vi "VarMan Spy.vi"() -> ()   [LabVIEW 2021]
doc: "VarMan Spy monitors VarMan's objects and allows performing some manipulations on them. Use a \"Spy\" menu to control the Spy.\nFor more information, see online help for the Spy.\n\n::: CalcExpress Toolkit :::\nCopyright (c) 2000-2026 Konstantin Shifershteyn. All rights reserved."
uses:
  _VarMan Spy.llb/VM Spy Type - Display Mode Selector.ctl
  <vilib>/Utility/sysdir.llb/System Directory Type.ctl
  <vilib>/Utility/miscctls.llb/LVRowAndColumnUnsignedTypeDef.ctl
  vi.lib/addons/CalcExpress/cemisc.llb/[ce] CE component paths - Kind of Path Enum.ctl
  <vilib>/Utility/config.llb/NI_LVConfig.lvlib
panel:
  in  "EnaFilter":bool=TRUE caption="Name filter"
  in  "NamePtrn":string caption="Name pattern"
  in  "VarList Mode":T1 caption="Display mode"
  in  "VC List":i32(listbox)=-1 caption="Context List"
  out "ctx info line":string caption="Context creator"
  in  "MaxWriteTS":dbl
  in  "Var List":i32[](listbox) caption="Variable List"
  out "var info line":string caption="info line"
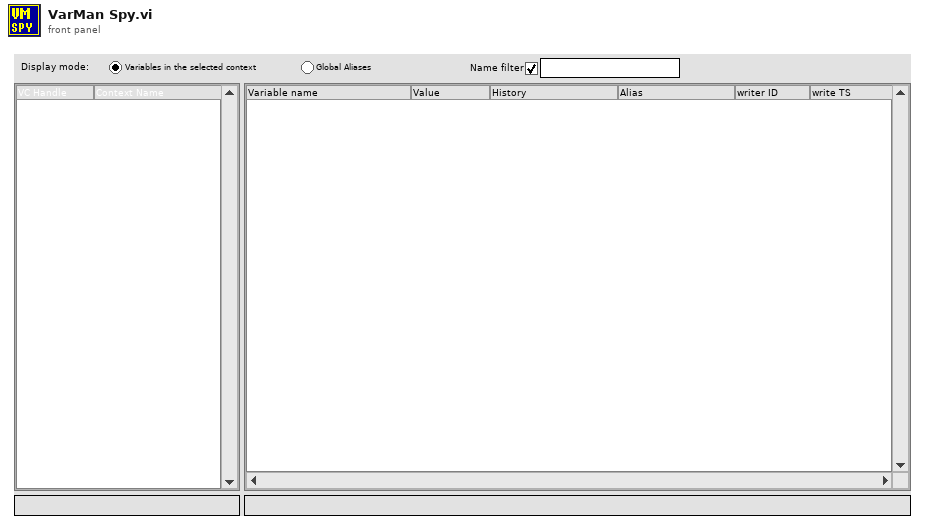
[diagram p1: front panel]
types:
  T1 = typedef "VM Spy Type - Display Mode Selector.ctl" = enum32{"Variables", "Aliases"}
  T2 = typedef "System Directory Type.ctl" = i32
  T3 = enum32{"invalid OS target", "Mac OS", "Windows 3.1", "Windows 95/NT", "Solaris 1", "Solaris 2", "HP-UX", "PowerMAX", "Linux", "Irix", "Rhapsody", "BeOS", "AIX", "OSF1", "VxWorks", "PharLap", "Carbon", "RTX", "Windows x64", "Linux x64", "Mac OS X x64"}
  T4 = typedef "LVRowAndColumnUnsignedTypeDef.ctl" = cluster{"Row":u32, "Column":u32}
  T5 = enum16{"don't sort", "alias", "vc handle", "name", "type"}
  T6 = typedef "VarMan Variable Context Handle.ctl" = i32
  T7 = typedef "VarMan Variable Info Cluster.ctl" = cluster{"name":string, "alias":string, "type":u32, "history":bool}
  T8 = cluster{"dup VC Handle":T6, "variables info":T7[]}
  T9 = typedef "VarMan Variable Data Statistics.ctl" = cluster{"writer ID":u32, "write MS":u32, "write TS":dbl, "write Cnt":u32}
  T10 = typedef "VarMan Alias Info Cluster.ctl" = cluster{"alias":string, "vc handle":T6, "var name":string, "type":u32, "history":bool}
  T11 = enum32{"invalid app kind", "Development System", "Run Time System", "Student Edition", "Embedded LabVIEW", "Evaluation", "Custom"}
  T12 = enum32{"Invalid", "Standard", "Closed", "Hidden", "Minimized", "Maximized"}
  T13 = typedef "[ce] CE component paths - Kind of Path Enum.ctl" = enum16{"VIs", "FuncVIs", "Help", "Examples", "Project", "Templates"}
  T14 = typedef "eventvkey.ctl" = enum16{"ASCII", "Enter", "Return", "Shift", "Ctrl", "Alt", "Cmd", "Opt", "Caps", "NumLock", "Clear", "Break", "Up", "Down", "Left", "Right", "Insert", "Delete", "Home", "End", "PageUp", "PageDown", "Escape", "Help", "Pause", "ScrollLock", "F1", "F2", "F3", "F4", "F5", "F6", "F7", "F8", "F9", "F10", "F11", "F12", "F13", "F14", "F15", "F16", "F17", "F18", "F19", "F20", "F21", "F22", "F23", "F24", "Play", "VolumeUp", "VolumeDown", "Mute", "Two Byte Char"}
  T15 = cluster{"Shift":bool, "Ctrl":bool, "Alt":bool, "Cmd":bool, "Opt":bool}
  T16 = typedef "LVPoint32TypeDef.ctl" = cluster{"Horizontal":i32, "Vertical":i32}
  T17 = typedef "LVRowAndColumnTypeDef.ctl" = cluster{"Row":i32, "Column":i32}
  T18 = typedef "NI_LVConfig.lvlib/Config Data RefNum.ctl" = refnum<k1>
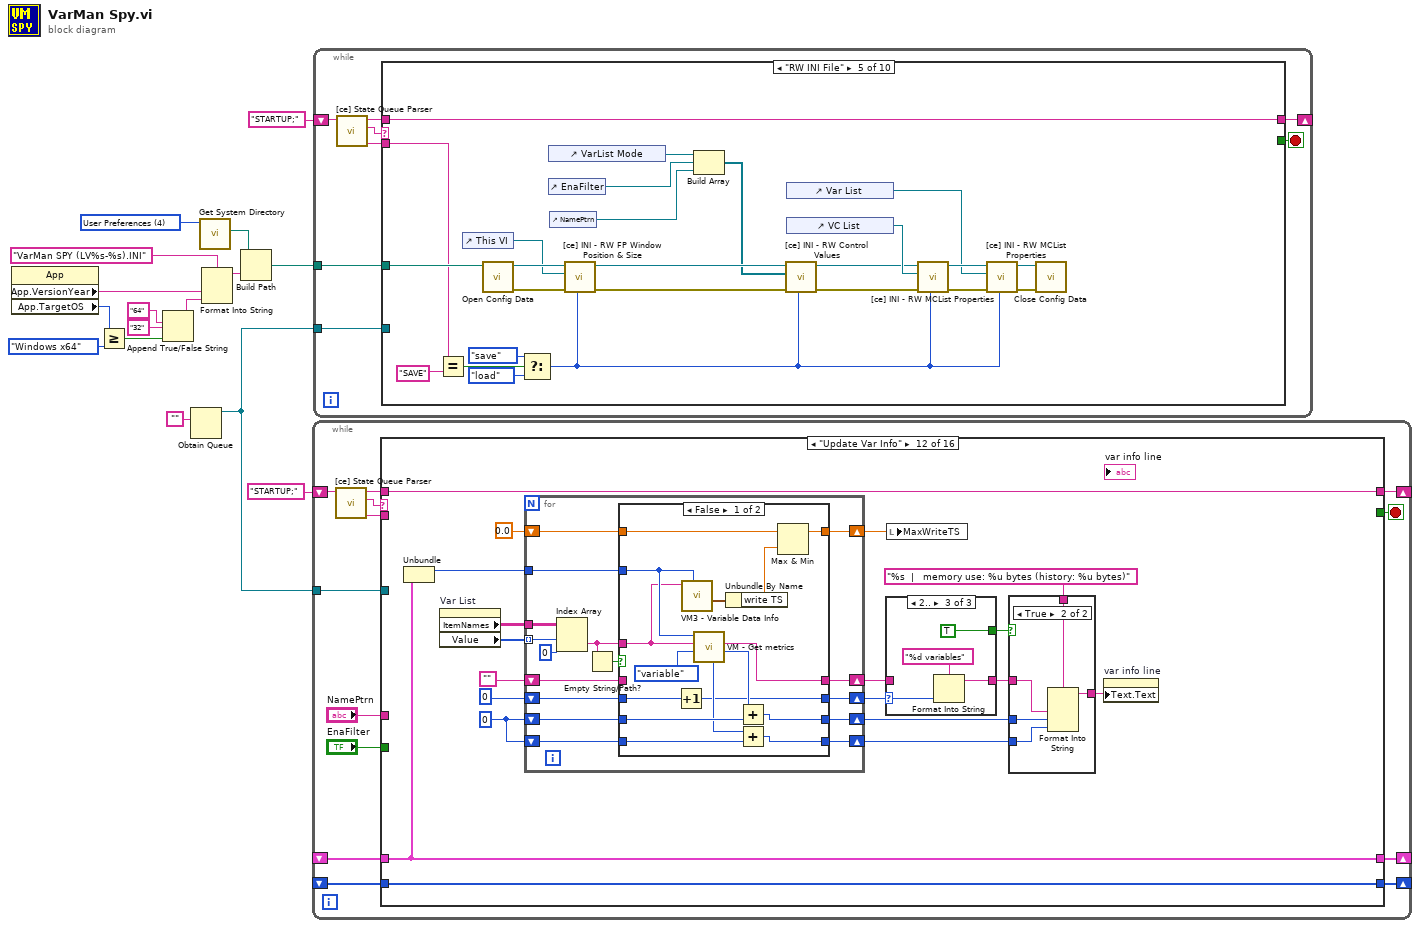
[diagram p0: block diagram]
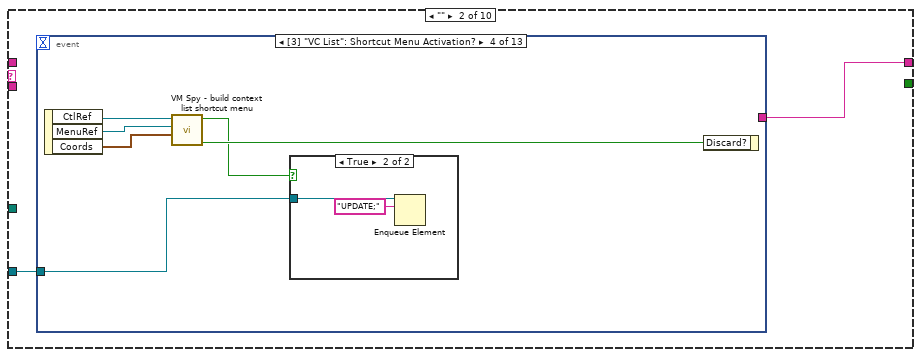
[diagram p3: hidden frame]
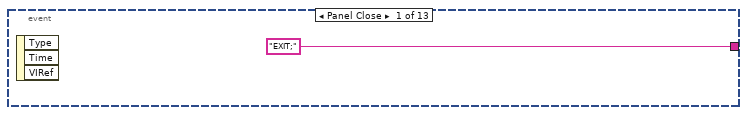
[diagram p4: hidden frame]
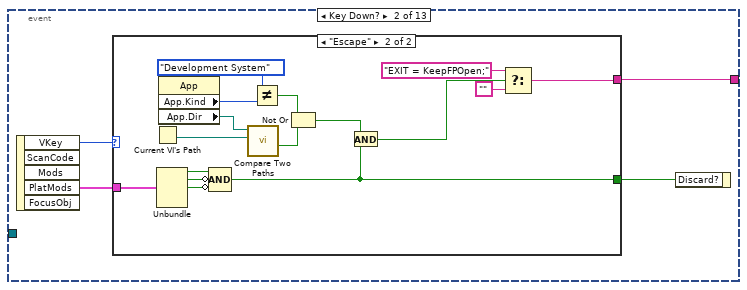
[diagram p5: hidden frame]
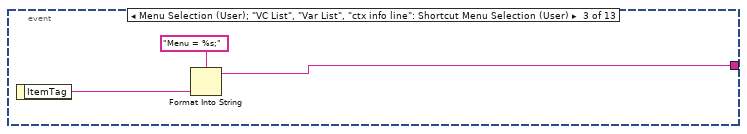
[diagram p7: hidden frame]
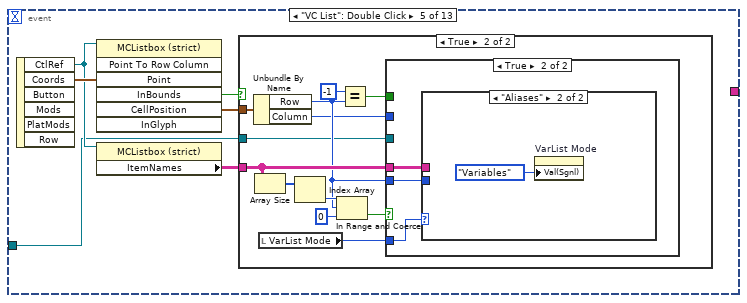
[diagram p9: hidden frame]
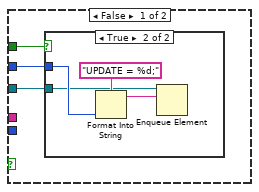
[diagram p11: hidden frame]
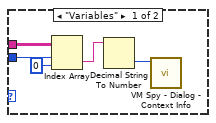
[diagram p13: hidden frame]
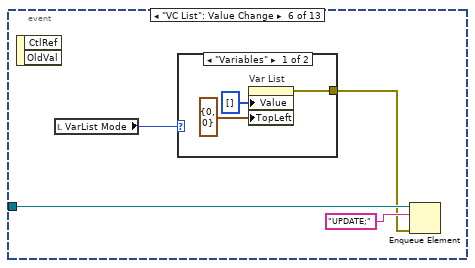
[diagram p14: hidden frame]
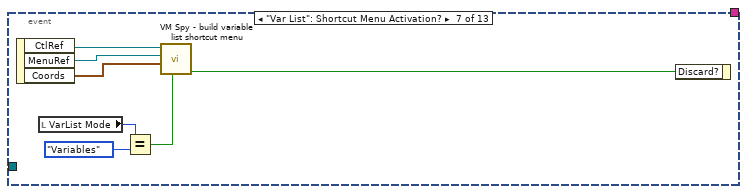
[diagram p16: hidden frame]
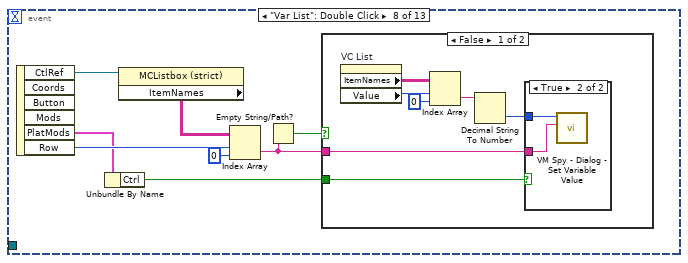
[diagram p17: hidden frame]
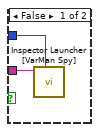
[diagram p18: hidden frame]
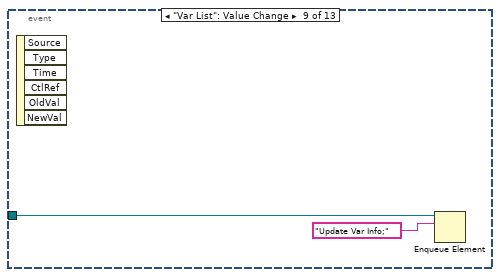
[diagram p20: hidden frame]
diagram:
  w2 = T2 4 items=["User Home"=0, "User Desktop"=1, "User Documents"=2, "User Application Data"=3, "User Preferences"=4, "User Temporary"=5, "Public Documents"=6, "Public Application Data"=7, "Public Preferences"=8, "Public Cache"=13, "System Core Libraries"=9, "System Installed Libraries"=10, "Application Files"=11, "Boot Volume Root"=12] ("system directory type")
  n1 = property class="App"() -> ("App.VersionYear"=w12:string, "App.TargetOS"=w10:T3)  [unwired: 2 in, 2 out]
  n2 = Greater Or Equal?(x=w10, y=T3."Windows x64" ("Application:Target:Operating System")) -> (x >= y?=w11:bool)
  n3 = Append True/False String(1:w11, 2:"32", 3:"64") -> (0:w9:string)  [unwired: 1 in]
  n4 = Obtain Queue(element data type="") -> (queue out=w13:refnum<queue>)  [unwired: 4 in, 2 out]
  n5 = call <vilib>:"Get System Directory.vi"("system directory type"=w2) -> ("system directory"=w8:path)  [unwired: 10 in]
  n6 = Format Into String(format string="VarMan SPY (LV%s-%s).INI", w12, w9) -> (resulting string=w7:string)  [unwired: 2 in, 1 out]
  n7 = Build Path(base path=w8, name or relative path=w7) -> (appended path=w1:path)
  n8 = while {
    shift-right: [w27] -> _
    shift-left: "STARTUP;" -> [w28]
    tunnel: w13 -> [w24]
    shift-right: [w21] -> _
    shift-left: _ -> [w20]
    shift-right: [w22] -> _
    shift-left: _ -> [w19]
    stop <- w25 stop-if-true
    n9 = call "[ce] State Queue Parser.vi"("input queue"=w28) -> ("state parameters"=w23:string, "state"=w29:string, "remained queue"=w26:string)  [unwired: 6 in]
    n10 = case shown="\"Update Var Info\"" w29 {
      tunnel: [w32 w43 w54 w59 w64 w71 w74 w98 w126 w142 w280 w385 w441 w444 w453 w457] -> w27
      tunnel: w26 -> [w32 _ w55 w60 w65 w71 w74 w99 w126 w149 w290 w385 w441 w444 w453 w464]
      tunnel: [_ _ _ _ _ TRUE _ _ _ _ _ _ _ _ _ _] -> w25
      tunnel: w24 -> [_ w50 _ _ _ w66 _ _ _ _ _ _ _ _ _ _]
      tunnel: w23 -> [_ _ _ _ _ _ _ w94 w117 w134 w272 _ _ _ w449 w460]
      tunnel: [w31 w34 w52 w57 w62 w69 w73 w97 w114 w147 w288 w382 w439 w443 w454 w465] -> w22
      tunnel: [w30 w33 w51 w56 w61 w68 w72 w96 w113 w148 w289 w384 w440 w442 w455 w459] -> w21
      tunnel: w20 -> [w30 w33 w51 w56 w61 w68 w72 w96 w112 w148 w289 w384 w440 w442 w455 w459]
      tunnel: w19 -> [w31 w34 w52 w57 w62 w69 w73 w97 _ w147 w288 w382 w439 w443 w454 w465]
      tunnel: "NamePtrn" -> [_ _ _ _ _ _ _ _ _ w132 w270 _ _ _ _ _]
      tunnel: "EnaFilter" -> [_ _ _ _ _ _ _ _ _ w131 w264 _ w438 _ _ _]
      frame Default {
      }
      frame "" {
        n11 = Dequeue Element(queue=w50, timeout in ms (-1)=100) -> (element=w47:string, error out=w46:errorcluster)  [unwired: 1 in, 2 out]
        n12 = Tick Count (ms)() -> (millisecond timer value=w42:u32)
        n13 = Quotient & Remainder(x=w42, y=u32 500) -> (floor(x/y)=w39:u32)  [unwired: 1 out]
        n14 = feedback-in #1(w39) -> ()
        n15 = feedback #1() -> (w40:u32)  [unwired: 1 in]
        n16 = Not Equal?(x=w39, y=w40) -> (x != y?=w38:bool)
        n17 = Select(t="UPDATE;", s=w38, f="") -> (s? t:f=w35:string)
        n18 = Empty String/Path?(string/path=w47) -> (empty?=w48:bool)
        n19 = Select(t=w35, s=w48, f=w47) -> (s? t:f=w45:string)
        n20 = Select(t="EXIT;", s=w46, f=w45) -> (s? t:f=w43:string)
      }
      frame "STARTUP" {
        n21 = Concatenate Strings("INIT;", w55) -> (w54:string)
      }
      frame "INIT" {
        n22 = Concatenate Strings("", w60) -> (w59:string)
      }
      frame "EXIT" {
        n23 = Concatenate Strings("HALT;", w65) -> (w64:string)
      }
      frame "HALT" {
        n24 = Release Queue(queue=w66, force destroy? (F)=TRUE) -> ()  [unwired: 1 in, 3 out]
      }
      frame "------------------------------------ 1" {
      }
      frame "UPDATE" {
        n25 = feedback-in #2("VarList Mode") -> ()
        n26 = feedback #2() -> (w93:T1)  [unwired: 1 in]
        n27 = First Call?() -> (First Call?: T/F=w91:bool)
        n28 = Not Equal?(x="VarList Mode", y=w93) -> (x != y?=w92:bool)
        n29 = Or(x=w92, y=w91) -> (x .or. y?=w90:bool)
        n30 = case shown="True" w90 {
          tunnel: "VarList Mode" -> [_ w103]
          tunnel: [_ TRUE] -> w88
          frame False {
          }
          frame True {
            n31 = case shown="\"Variables\"" w103 {
              tunnel: [string[] ["Variable name", "Value", "History", "Alias", "writer ID", "write TS"] ("Column Header Strings[]") string[] ["Alias", "Value", "History", "Variable", "writer ID", "write TS"] ("Column Header Strings[]")] -> w104
              frame "Variables" {
              }
              frame "Aliases" {
              }
            }
            n32 = property on="Var List" class="MCListbox (strict)"("ColHdrString"=w104, "TopLeft"=T4 {"Row"=0, "Column"=0} ("Top Left Visible Cell"), "Value"=i32[] [] ("Var List")) -> ()  [unwired: 2 in, 2 out]
          }
        }
        n33 = case shown="\"Aliases\"" "VarList Mode" {
          tunnel: ["Update Var List = %s;" "Update Alias List = %s;"] -> w79
          frame "Variables" {
          }
          frame "Aliases" {
          }
        }
        n34 = Format Into String(format string="Update VC List = %s;", w94) -> (resulting string=w81:string)  [unwired: 2 in, 1 out]
        n35 = feedback #3(u32 0) -> (w86:u32)
        n36 = Increment(x=w86) -> (x+1=w84:u32)
        n37 = feedback-in #3(w84) -> ()
        n38 = Quotient & Remainder(x=w84, y=u32 20) -> (x-y*floor(x/y)=w82:u32)  [unwired: 1 out]
        n39 = Equal To 0?(x=w82) -> (x = 0?=w87:bool)
        n40 = Or(x=w87, y=w88) -> (x .or. y?=w78:bool)
        n41 = Select(t="MAX", s=w78, f="") -> (s? t:f=w76:string)
        n42 = Format Into String(format string=w79, w76) -> (resulting string=w80:string)  [unwired: 2 in, 1 out]
        n43 = Concatenate Strings(w81, w80, w99) -> (w98:string)
      }
      frame "Update VC List" {
        n44 = Decimal String To Number(string=w117, default (0L)=-1 ("default (0 I32)")) -> (number=w115:i32)  [unwired: 1 in, 1 out]
        n45 = control-ref of="VC List"() -> (w120:refnum<vi>)
        n46 = Index Array(array=w112, index="VC List") -> (element=w122:T6)
        n47 = call "VM Spy - build list of contexts.vi"("sort column"=w115, "MCListbox Refnum"=w120) -> ("array of VC handles"=w113:T6[], "dup MCListbox Refnum"=w119:refnum<vi>)  [unwired: 5 in, 1 out]
        n48 = Search 1D Array(1D array=w113, element=w122) -> (index of element=w121:i32)  [unwired: 1 in]
        n49 = Not Equal?(x=w121, y="VC List") -> (x != y?=w123:bool)
        n50 = Index Array(array=w113, index=w121) -> (element=w118:T6)
        n51 = case shown="True" w123 {
          tunnel: w121 -> [_ w128]
          tunnel: w119 -> [_ w127]
          frame False {
          }
          frame True {
            n52 = local write "VC List"(w128) -> ()
            n53 = call "VM Spy - MCListBox make row visible.vi"("visible row"=w128, "MCListbox Refnum"=w127) -> ()  [unwired: 6 in, 2 out]
          }
        }
        n54 = call "VM - Context Info.vi"("VC Handle"=w118) -> ("Creator"=→"ctx info line":string)  [unwired: 6 in, 4 out]
        n55 = call "VM - List of Variables.vi"("sort"=enum16{"don't sort", "name", "alias", "type"}."name", "VC Handle"=w118) -> ("variables info"=w125:T7[], "dup VC Handle"=w124:T6)  [unwired: 5 in, 1 out]
        n56 = Bundle("dup VC Handle"=w124, "variables info"=w125) -> (w114:T8)  [unwired: 1 in]
      }
      frame "Update Var List" {
        n57 = Unbundle(w147) -> ("dup VC Handle"=w143:T6, "variables info"=w137:T7[])
        n58 = Empty String/Path?(string/path=w132) -> (empty?=w133:bool)
        n59 = Compound Arithmetic op=OR(w133, invert w131) -> (w130:bool)
        n60 = for {
          tunnel: w137 -> [w193] mode=indexing
          tunnel: w143 -> [w189]
          tunnel: [w191] -> w146 mode=indexing if=w185
          tunnel: [w190] -> w145 mode=indexing if=w185
          tunnel: [w187] -> w138 mode=indexing if=w185
          tunnel: w132 -> [w182]
          tunnel: w130 -> [w181]
          n61 = Unbundle By Name(w193) -> ("alias"=w184:string, "history"=w188:bool, "name"=w183:string, "type"=w192:u32)
          n62 = case shown="False" w181 {
            selector: w181 -> [_ w198]
            tunnel: [w196 w198] -> w186
            tunnel: w183 -> [w195 _]
            tunnel: w182 -> [w194 _]
            frame False {
              n63 = Match Pattern(string=w195, regular expression=w194) -> (offset past match=w197:i32)  [unwired: 1 in, 3 out]
              n64 = Greater Or Equal To 0?(x=w197) -> (x >= 0?=w196:bool)
            }
            frame True {
            }
          }
          n65 = case shown="True" w186 {
            tunnel: w192 -> [_ w215]
            tunnel: w184 -> [_ w213]
            tunnel: [_ w212] -> w191
            tunnel: [_ w211] -> w190
            tunnel: w189 -> [_ w210]
            tunnel: w183 -> [_ w209]
            tunnel: w188 -> [_ w204]
            tunnel: [_ w200] -> w187
            tunnel: [_ TRUE] -> w185
            frame False {
            }
            frame True {
              n66 = case shown="1" w215 {
                selector: w215 -> [_ _ _ _ _ _ w258]
                tunnel: w209 -> [w219 w226 w233 w236 w244 w249 w253]
                tunnel: w210 -> [w217 w225 w232 w235 w242 w248 w252]
                tunnel: ["..." w222 w229 w238 "[..]" "[[..]]" w260] -> w214
                tunnel: [w218 w224 w231 w240 w243 w247 w261] -> w205
                tunnel: [w216 w221 w227 w234 w241 w246 w251] -> w206
                frame Default {
                  n67 = call "VM3 - Variable Data Info.vi"("VC Handle"=w217, "name_spec"=w219) -> ("stats"=w216:T9, "dup name_spec"=w218:string)  [unwired: 4 in, 4 out]
                }
                frame 0 {
                  n68 = call "VM3 - String.vi"("VC Handle"=w225, "name_spec"=w226) -> ("stats"=w221:T9, "value out"=w223:string, "dup name_spec"=w224:string)  [unwired: 6 in, 1 out]
                  n69 = call "VM Spy - Truncate string value for list.vi"("String in"=w223) -> ("String out"=w222:string)  [unwired: 10 in]
                }
                frame 1 {
                  n70 = call "VM3 - DBL Scalar.vi"("VC Handle"=w232, "name_spec"=w233) -> ("stats"=w227:T9, "value out"=w230:dbl, "dup name_spec"=w231:string)  [unwired: 6 in, 1 out]
                  n71 = Format Value(format string="%.;%#_9g", value (0)=w230) -> (output string=w229:string)  [unwired: 1 in]
                }
                frame 5 {
                  n72 = call "VM3 - CDB Scalar.vi"("VC Handle"=w235, "name_spec"=w236) -> ("stats"=w234:T9, "value out"=w239:cdb, "dup name_spec"=w240:string)  [unwired: 6 in, 1 out]
                  n73 = Format Value(format string="%.;%#_g", value (0)=w239) -> (output string=w238:string)  [unwired: 1 in]
                }
                frame 3, 6, 8 {
                  n74 = call "VM3 - Variable Data Info.vi"("VC Handle"=w242, "name_spec"=w244) -> ("stats"=w241:T9, "dup name_spec"=w243:string)  [unwired: 4 in, 4 out]
                }
                frame 4, 7, 9 {
                  n75 = call "VM3 - Variable Data Info.vi"("VC Handle"=w248, "name_spec"=w249) -> ("stats"=w246:T9, "dup name_spec"=w247:string)  [unwired: 4 in, 4 out]
                }
                frame 252 {
                  n76 = call "VM3 - Arbitrary Data.vi"("var type in"=w258, "VC Handle"=w252, "name_spec"=w253) -> ("stats"=w251:T9, "flattened value out"=w257:string, "dup name_spec"=w261:string)  [unwired: 4 in, 2 out]
                  n77 = call "[ce] Index Range from Flattened String.vi"("Flattened string"=w257) -> ("Index Range"=w256:cluster{"Initial index":i32, "Final index":i32})  [unwired: 10 in]
                  n78 = Unbundle(w256) -> ("Initial index"=w254:i32, "Final index"=w255:i32)
                  n79 = Format Into String(format string="{%d:%d}", w254, w255) -> (resulting string=w260:string)  [unwired: 2 in, 1 out]
                }
              }
              n80 = call "VM Spy - VM Datatype to List Symbol.vi"("VarMan Datatype Code"=w215) -> ("List/Tree Symbol"=w211:i32)  [unwired: 10 in]
              n81 = Unbundle By Name(w206) -> ("writer ID"=w207:u32, "write TS"=w200:dbl)
              n82 = call "VM Spy - format history info for variable list.vi"("Has history"=w204, "Variable name"=w205, "VC Handle"=w210) -> ("String out"=w208:string)  [unwired: 8 in]
              n83 = Number To Decimal String(number=w207) -> (decimal integer string=w203:string)  [unwired: 1 in]
              n84 = Format Date/Time String(time format string (%c)="%X%3u %x", seconds (now)=w200) -> (date/time string=w202:string)  [unwired: 1 in]
              n85 = Build Array(w205, w214, w208, w213, w203, w202) -> (w212:string[])
            }
          }
        }
        n86 = feedback-in #4(w143) -> ()
        n87 = feedback #4() -> (w144:T6)  [unwired: 1 in]
        n88 = Not Equal?(x=w143, y=w144) -> (x != y?=w136:bool)
        n89 = case shown="False" w136 {
          tunnel: w146 -> [w154 w169]
          tunnel: w145 -> [w153 w160]
          tunnel: w138 -> [_ w168]
          tunnel: [TRUE w167] -> w135
          tunnel: w134 -> [_ w161]
          frame True {
            n90 = property on="Var List" class="MCListbox (strict)"("TopLeft"=T4 {"Row"=0, "Column"=0} ("Top Left Visible Cell"), "Value"=i32[] [] ("Var List"), "ItemNames"=w154, "ItemSyms"=w153) -> ()  [unwired: 2 in, 2 out]
          }
          frame False {
            n91 = Array Size(array=w160) -> (size(s)=w164:i32)
            n92 = property on="Var List" class="MCListbox (strict)"("ItemNames"=w169, "ItemSyms"=w160) -> ("Value"=w158:i32[])  [unwired: 2 in, 2 out]
            n93 = feedback #5() -> (w163:i32)  [unwired: 1 in]
            n94 = feedback-in #5(w164) -> ()
            n95 = Empty Array?(array=w158) -> (empty?=w157:bool)
            n96 = Not Equal?(x=w164, y=w163) -> (x != y?=w156:bool)
            n97 = Equal?(x=w161, y="MAX") -> (x = y?=w165:bool)
            n98 = And(x=w157, y=w156) -> (x .and. y?=w155:bool)
            n99 = Or(x=w156, y=w165) -> (x .or. y?=w159:bool)
            n100 = case shown="True" w155 {
              frame False {
              }
              frame True {
                n101 = property on="Var List" class="MCListbox (strict)"("TopLeft"=T4 {"Row"=0, "Column"=0} ("Top Left Visible Cell")) -> ()  [unwired: 2 in, 2 out]
              }
            }
            n102 = case shown="False" w159 {
              selector: w159 -> [_ w180]
              tunnel: w158 -> [w174 _]
              tunnel: w168 -> [w173 _]
              tunnel: "MaxWriteTS" -> [w172 _]
              tunnel: [w171 w180] -> w167
              frame False {
                n103 = for {
                  tunnel: w174 -> [w179] mode=indexing
                  tunnel: w173 -> [w178]
                  tunnel: w172 -> [w176]
                  tunnel: [w175] -> w171
                  stop <- w175 stop-if-true
                  n104 = Index Array(array=w178, index=w179) -> (element=w177:dbl)
                  n105 = Greater?(x=w177, y=w176) -> (0:w175:bool)
                }
              }
              frame True {
              }
            }
          }
        }
        n106 = Select(t="Update Var Info;", s=w135, f="") -> (s? t:f=w140:string)
        n107 = Concatenate Strings("Update UI Properties;", w140, w149) -> (w142:string)
      }
      frame "Update Alias List" {
        n108 = Empty String/Path?(string/path=w270) -> (empty?=w265:bool)
        n109 = call "VM - List of Aliases.vi"("sort"=T5."alias") -> ("aliases info"=w282:T10[])  [unwired: 9 in, 1 out]
        n110 = Compound Arithmetic op=OR(w265, invert w264) -> (w263:bool)
        n111 = for {
          tunnel: w282 -> [w315] mode=indexing
          tunnel: [w313] -> w287 mode=indexing if=w307
          tunnel: [w312] -> w271 mode=indexing if=w307
          tunnel: [w308] -> w285 mode=indexing if=w307
          tunnel: w270 -> [w306]
          tunnel: w263 -> [w303]
          n112 = Unbundle By Name(w315) -> ("alias"=w304:string, "history"=w309:bool, "vc handle"=w310:T6, "var name"=w311:string, "type"=w314:u32)
          n113 = case shown="False" w303 {
            selector: w303 -> [_ w366]
            tunnel: w306 -> [w365 _]
            tunnel: [w363 w366] -> w305
            tunnel: w304 -> [w362 _]
            frame False {
              n114 = Match Pattern(string=w362, regular expression=w365) -> (offset past match=w364:i32)  [unwired: 1 in, 3 out]
              n115 = Greater Or Equal To 0?(x=w364) -> (x >= 0?=w363:bool)
            }
            frame True {
            }
          }
          n116 = case shown="True" w305 {
            tunnel: w314 -> [_ w336]
            tunnel: [_ w334] -> w313
            tunnel: [_ w333] -> w312
            tunnel: w311 -> [_ w325]
            tunnel: w304 -> [_ w323]
            tunnel: w310 -> [_ w322]
            tunnel: w309 -> [_ w321]
            tunnel: [_ w317] -> w308
            tunnel: [_ TRUE] -> w307
            frame False {
            }
            frame True {
              n117 = case shown="1" w336 {
                tunnel: w325 -> [w340 w347 w354 w356]
                tunnel: w322 -> [w338 w346 w353 w357]
                tunnel: ["..." w343 w350 w359] -> w335
                tunnel: [w339 w345 w352 w361] -> w324
                tunnel: [w337 w342 w348 w355] -> w326
                frame Default {
                  n118 = call "VM3 - Variable Data Info.vi"("VC Handle"=w338, "name_spec"=w340) -> ("stats"=w337:T9, "dup name_spec"=w339:string)  [unwired: 4 in, 4 out]
                }
                frame 0 {
                  n119 = call "VM3 - String.vi"("VC Handle"=w346, "name_spec"=w347) -> ("stats"=w342:T9, "value out"=w344:string, "dup name_spec"=w345:string)  [unwired: 6 in, 1 out]
                  n120 = call "VM Spy - Truncate string value for list.vi"("String in"=w344) -> ("String out"=w343:string)  [unwired: 10 in]
                }
                frame 1 {
                  n121 = call "VM3 - DBL Scalar.vi"("VC Handle"=w353, "name_spec"=w354) -> ("stats"=w348:T9, "value out"=w351:dbl, "dup name_spec"=w352:string)  [unwired: 6 in, 1 out]
                  n122 = Format Value(format string="%.;%#_9g", value (0)=w351) -> (output string=w350:string)  [unwired: 1 in]
                }
                frame 5 {
                  n123 = call "VM3 - CDB Scalar.vi"("VC Handle"=w357, "name_spec"=w356) -> ("stats"=w355:T9, "value out"=w360:cdb, "dup name_spec"=w361:string)  [unwired: 6 in, 1 out]
                  n124 = Format Value(format string="%.;%#_g", value (0)=w360) -> (output string=w359:string)  [unwired: 1 in]
                }
              }
              n125 = call "VM Spy - VM Datatype to List Symbol.vi"("VarMan Datatype Code"=w336) -> ("List/Tree Symbol"=w333:i32)  [unwired: 10 in]
              n126 = Unbundle By Name(w326) -> ("writer ID"=w327:u32, "write TS"=w317:dbl)
              n127 = Concatenate Strings("=" ("string"), w323) -> (w332:string)
              n128 = call "VM Spy - format history info for variable list.vi"("Has history"=w321, "Variable name"=w324, "VC Handle"=w322) -> ("String out"=w328:string)  [unwired: 8 in]
              n129 = Format Into String(format string=" (VC:%d)", initial string=w324, w322) -> (resulting string=w329:string)  [unwired: 1 in, 1 out]
              n130 = Number To Decimal String(number=w327) -> (decimal integer string=w320:string)  [unwired: 1 in]
              n131 = Format Date/Time String(time format string (%c)="%X%3u %x", seconds (now)=w317) -> (date/time string=w319:string)  [unwired: 1 in]
              n132 = Build Array(w332, w335, w328, w329, w320, w319) -> (w334:string[])
            }
          }
        }
        n133 = Array Size(array=w271) -> (size(s)=w283:i32)
        n134 = property on="Var List" class="MCListbox (strict)"("ItemNames"=w287, "ItemSyms"=w271) -> ("Value"=w267:i32[])  [unwired: 2 in, 2 out]
        n135 = feedback #6() -> (w284:i32)  [unwired: 1 in]
        n136 = feedback-in #6(w283) -> ()
        n137 = local read "MaxWriteTS"() -> (w281:dbl)
        n138 = Empty Array?(array=w267) -> (empty?=w269:bool)
        n139 = Not Equal?(x=w283, y=w284) -> (x != y?=w266:bool)
        n140 = Equal?(x=w272, y="MAX") -> (x = y?=w276:bool)
        n141 = And(x=w269, y=w266) -> (x .and. y?=w268:bool)
        n142 = Or(x=w266, y=w276) -> (x .or. y?=w275:bool)
        n143 = case shown="False" w275 {
          selector: w275 -> [_ w302]
          tunnel: w285 -> [w295 _]
          tunnel: w267 -> [w294 _]
          tunnel: w281 -> [w293 _]
          tunnel: [w292 w302] -> w274
          tunnel: w268 -> [w291 _]
          frame False {
            n144 = case shown="True" w291 {
              frame False {
              }
              frame True {
                n145 = property on="Var List" class="MCListbox (strict)"("TopLeft"=T4 {"Row"=0, "Column"=0} ("Top Left Visible Cell")) -> ()  [unwired: 2 in, 2 out]
              }
            }
            n146 = for {
              tunnel: w294 -> [w301] mode=indexing
              tunnel: w295 -> [w300]
              tunnel: w293 -> [w298]
              tunnel: [w297] -> w292
              stop <- w297 stop-if-true
              n147 = Index Array(array=w300, index=w301) -> (element=w299:dbl)
              n148 = Greater?(x=w299, y=w298) -> (0:w297:bool)
            }
          }
          frame True {
          }
        }
        n149 = Select(t="Update Var Info;", s=w274, f="") -> (s? t:f=w277:string)
        n150 = Concatenate Strings("Update UI Properties;", w277, w290) -> (w280:string)
      }
      frame "Update Var Info" {
        w379 = u64 0
        n151 = Unbundle(w382) -> ("dup VC Handle"=w373:T6)  [unwired: 1 out]
        n152 = property on="Var List" class="MCListbox (strict)"() -> ("ItemNames"=w383:string[][], "Value"=w380:i32[])  [unwired: 2 in, 2 out]
        n153 = for {
          tunnel: w383 -> [w413]
          tunnel: w380 -> [w412] mode=indexing
          shift-right: [w410] -> w378
          shift-left: w379 -> [w409]
          shift-right: [w408] -> w377
          shift-left: w379 -> [w407]
          shift-right: [w404] -> w370
          shift-left: "" -> [w403]
          shift-right: [w402] -> w372
          shift-left: 0 -> [w401]
          tunnel: w373 -> [w400]
          shift-right: [w398] -> w367
          shift-left: 0.0 -> [w399]
          n154 = Index Array(array=w413, index (row)=w412, index (col)=0 ("disabled index (col)")) -> (element=w405:string)
          n155 = Empty String/Path?(string/path=w405) -> (empty?=w406:bool)
          n156 = case shown="False" w406 {
            tunnel: w405 -> [w418 _]
            tunnel: [w427 w434] -> w410
            tunnel: w409 -> [w426 w434]
            tunnel: [w424 w433] -> w408
            tunnel: w407 -> [w423 w433]
            tunnel: w400 -> [w419 _]
            tunnel: [w422 w432] -> w404
            tunnel: w403 -> [_ w432]
            tunnel: [w420 w431] -> w402
            tunnel: w401 -> [w421 w431]
            tunnel: w399 -> [w416 w430]
            tunnel: [w415 w430] -> w398
            frame False {
              n157 = Increment(x=w421) -> (x+1=w420:i32)
              n158 = call "VM3 - Variable Data Info.vi"("VC Handle"=w419, "name_spec"=w418) -> ("stats"=w417:T9)  [unwired: 4 in, 5 out]
              n159 = call "VM - Get metrics.vi"("object"=enum32{"variable", "context", "total"}."variable", "name spec"=w418, "VC Handle"=w419) -> ("total size, bytes"=w428:u64, "dup name spec"=w422:string, "history size, bytes"=w425:u64)  [unwired: 4 in, 2 out]
              n160 = Unbundle By Name(w417) -> ("write TS"=w414:dbl)
              n161 = Add(x=w428, y=w426) -> (x+y=w427:u64)
              n162 = Add(x=w425, y=w423) -> (x+y=w424:u64)
              n163 = Max & Min(x=w416, y=w414) -> (max(x,y)=w415:dbl)  [unwired: 1 out]
            }
            frame True {
            }
          }
        }
        n164 = case shown="2.." w372 {
          selector: w372 -> [_ _ w397]
          tunnel: [_ w393 w396] -> w371
          tunnel: w370 -> [_ w393 _]
          tunnel: [_ TRUE TRUE] -> w369
          frame ..0 {
          }
          frame 1 {
          }
          frame 2.. {
            n165 = Format Into String(format string="%d variables", w397) -> (resulting string=w396:string)  [unwired: 2 in, 1 out]
          }
        }
        n166 = local write "MaxWriteTS"(w367) -> ()
        n167 = case shown="True" w369 {
          tunnel: [w386 w391] -> w381
          tunnel: w378 -> [_ w390]
          tunnel: w377 -> [_ w389]
          tunnel: "%s  |   memory use: %u bytes (history: %u bytes)" -> [_ w388]
          tunnel: w371 -> [w386 w387]
          frame False {
          }
          frame True {
            n168 = Format Into String(format string=w388, w387, w390, w389) -> (resulting string=w391:string)  [unwired: 2 in, 1 out]
          }
        }
        n169 = property on="var info line" class="Str"("Text.Text"=w381) -> ()  [unwired: 2 in, 2 out]
      }
      frame "Update UI Properties" {
        n170 = Select(t=u32 16711680, s=w438, f=u32 0) -> (s? t:f=w435:u32)
        n171 = property on="NamePtrn" class="Str"("Text.FontColor"=w435) -> ()  [unwired: 2 in, 2 out]
      }
      frame "------------------------------------ 2" {
      }
      frame "Highlight Variable" {
        n172 = property on="Var List" class="MCListbox (strict)"() -> ("ItemNames"=w452:string[][])  [unwired: 2 in, 2 out]
        n173 = Index Array(array=w452, index (col)=0 ("disabled index (col)")) -> (element=w451:string[])  [unwired: 1 in]
        n174 = Search 1D Array(1D array=w451, element=w449) -> (index of element=w446:i32)  [unwired: 1 in]
        n175 = control-ref of="Var List"() -> (w448:refnum<vi>)
        n176 = Build Array(w446) -> (w445:i32[])
        n177 = property class="MCListbox (strict)"(reference=w448, "Value"=w445) -> (reference out=w447:refnum<vi>)  [unwired: 1 in, 1 out]
        n178 = call "VM Spy - MCListBox make row visible.vi"("visible row"=w446, "MCListbox Refnum"=w447) -> ()  [unwired: 6 in, 2 out]
      }
      frame "Highlight Context" {
        n179 = Decimal String To Number(string=w460) -> (number=w458:i32)  [unwired: 2 in, 1 out]
        n180 = Search 1D Array(1D array=w459, element=w458) -> (index of element=w461:i32)  [unwired: 1 in]
        n181 = control-ref of="VC List"() -> (w463:refnum<vi>)
        n182 = property class="MCListbox (strict)"(reference=w463, "Value"=w461) -> (reference out=w462:refnum<vi>)  [unwired: 1 in, 1 out]
        n183 = call "VM Spy - MCListBox make row visible.vi"("visible row"=w461, "MCListbox Refnum"=w462) -> ()  [unwired: 6 in, 2 out]
        n184 = Concatenate Strings("UPDATE;" ("string"), w464) -> (w457:string)
      }
    }
  }
  n185 = while {
    shift-right: [w471] -> _
    shift-left: "STARTUP;" -> [w472]
    tunnel: w13 -> [w468]
    tunnel: w1 -> [w466]
    stop <- w469 stop-if-true
    n186 = call "[ce] State Queue Parser.vi"("input queue"=w472) -> ("state parameters"=w467:string, "state"=w473:string, "remained queue"=w470:string)  [unwired: 6 in]
    n187 = case shown="\"RW INI File\"" w473 {
      tunnel: [w474 w476 w617 w624 w650 w653 w658 w659 w666 w685] -> w471
      tunnel: w470 -> [w474 _ w618 w625 w650 _ w658 w659 w666 w686]
      tunnel: [_ _ _ _ _ _ TRUE _ _ _] -> w469
      tunnel: w468 -> [_ w475 _ w620 _ w651 _ _ _ w669]
      tunnel: w467 -> [_ _ _ _ w642 w654 w656 _ _ w684]
      tunnel: w466 -> [_ _ _ _ w643 _ _ _ _ _]
      frame Default {
      }
      frame "" {
        n188 = event shown="[3] \"VC List\": Shortcut Menu Activation?" {
          selector: _ -> [_ _ _ _ _ _ _ _ _ _ _ _ _]
          dyn-events: _ -> [_ _ _ _ _ _ _ _ _ _ _ _ _]
          timeout: _ -> [_ _ _ _ _ _ _ _ _ _ _ _ _]
          tunnel: ["EXIT;" w480 w498 _ _ _ _ _ _ _ _ _ _] -> w476
          tunnel: w475 -> [_ _ _ w501 w509 w546 _ _ w576 w583 w588 w595 _]
          event Panel Close {
            n189 = event-data() -> ()  [unwired: 1 in, 3 out]
          }
          event Key Down? {
            n190 = event-data() -> ("VKey"=w478:T14, "PlatMods"=w481:T15)  [unwired: 1 in, 3 out]
            n191 = case shown="\"Escape\"" w478 {
              tunnel: w481 -> [_ w492]
              tunnel: [_ w491] -> w480
              tunnel: [_ w483] -> w479
              frame Default {
              }
              frame "Escape" {
                n192 = Current VI's Path() -> (path=w490:path)
                n193 = Unbundle(w492) -> ("Shift"=w495:bool, "Ctrl"=w494:bool, "Alt"=w493:bool)  [unwired: 2 out]
                n194 = property class="App"() -> ("App.Kind"=w488:T11, "App.Dir"=w489:path)  [unwired: 2 in, 2 out]
                n195 = Compound Arithmetic op=AND(w495, invert w494, invert w493) -> (w483:bool)
                n196 = call <vilib>:"Compare Two Paths.vi"("Path 2"=w490, "Path 1"=w489) -> ("Path 2 Relative to Path 1?"=w485:bool)  [unwired: 6 in, 3 out]
                n197 = Not Equal?(x=T11."Development System", y=w488) -> (x != y?=w486:bool)
                n198 = Not Or(1:w485, 2:w486) -> (0:w484:bool)
                n199 = And(x=w484, y=w483) -> (x .and. y?=w482:bool)
                n200 = Select(t="EXIT = KeepFPOpen;", s=w482, f="") -> (s? t:f=w491:string)
              }
            }
            n201 = event-data("Discard?"=w479) -> ()  [unwired: 1 in, 1 out]
          }
          event Menu Selection (User); "VC List", "Var List", "ctx info line": Shortcut Menu Selection (User) {
            n202 = event-data() -> ("ItemTag"=w500:string)  [unwired: 1 in]
            n203 = Format Into String(format string="Menu = %s;", w500) -> (resulting string=w498:string)  [unwired: 2 in, 1 out]
          }
          event "VC List": Shortcut Menu Activation? {
            n204 = event-data() -> ("CtlRef"=w506:refnum<vi>, "MenuRef"=w505:refnum<k9>, "Coords"=w504:T16)  [unwired: 1 in]
            n205 = call "VM Spy - build context list shortcut menu.vi"("Coords"=w504, "MenuRef"=w505, "CtlRef"=w506) -> ("Discard menu"=w503:bool, "Value changed"=w502:bool)  [unwired: 7 in]
            n206 = case shown="True" w502 {
              tunnel: w501 -> [_ w508]
              frame False {
              }
              frame True {
                n207 = Enqueue Element(queue=w508, element="UPDATE;") -> ()  [unwired: 2 in, 3 out]
              }
            }
            n208 = event-data("Discard?"=w503) -> ()  [unwired: 1 in, 1 out]
          }
          event "VC List": Double Click {
            n209 = event-data() -> ("CtlRef"=w511:refnum<vi>, "Coords"=w514:T16)  [unwired: 1 in, 4 out]
            n210 = invoke class="MCListbox (strict)" method="Point To Row Column"(reference=w511, "Point"=w514) -> ("InBounds"=w513:bool, "CellPosition"=w512:T17)  [unwired: 5 in, 5 out]
            n211 = property on="Property Node" class="MCListbox (strict)"(reference=w511) -> ("ItemNames"=w510:string[][])  [unwired: 1 in, 2 out]
            n212 = case shown="True" w513 {
              tunnel: w512 -> [_ w526]
              tunnel: w510 -> [_ w521]
              tunnel: w509 -> [_ w516]
              frame False {
              }
              frame True {
                n213 = Unbundle By Name(w526) -> ("Row"=w520:i32, "Column"=w517:i32)
                n214 = Array Size(array=w521) -> (size(s)=w523:i32[])
                n215 = local read "VarList Mode"() -> (w515:T1)
                n216 = Index Array(array=w523) -> (element=w524:i32)  [unwired: 1 in]
                n217 = In Range and Coerce(upper limit=w524, x=w520, lower limit=0) -> (In Range?=w522:bool)  [unwired: 1 out]
                n218 = Equal?(x=-1, y=w520) -> (x = y?=w518:bool)
                n219 = case shown="True" w522 {
                  tunnel: w521 -> [_ w536]
                  tunnel: w520 -> [_ w535]
                  tunnel: w518 -> [w529 _]
                  tunnel: w517 -> [w528 _]
                  tunnel: w516 -> [w527 _]
                  tunnel: w515 -> [_ w534]
                  frame False {
                    n220 = case shown="True" w529 {
                      tunnel: w528 -> [_ w531]
                      tunnel: w527 -> [_ w530]
                      frame False {
                      }
                      frame True {
                        n221 = Format Into String(format string="UPDATE = %d;" ("element"), w531) -> (resulting string=w532:string)  [unwired: 2 in, 1 out]
                        n222 = Enqueue Element(queue=w530, element=w532) -> ()  [unwired: 2 in, 3 out]
                      }
                    }
                  }
                  frame True {
                    n223 = case shown="\"Aliases\"" w534 {
                      tunnel: w536 -> [w541 _]
                      tunnel: w535 -> [w540 _]
                      frame "Variables" {
                        n224 = Index Array(array=w541, index (row)=w540, index (col)=0 ("disabled index (col)")) -> (element=w538:string)
                        n225 = Decimal String To Number(string=w538) -> (number=w537:i32)  [unwired: 2 in, 1 out]
                        n226 = call "VM Spy - Dialog - Context Info.vi"("VC Handle"=w537) -> ()  [unwired: 10 in, 1 out]
                      }
                      frame "Aliases" {
                        n227 = property on="VarList Mode" class="RadioBtnsControl (strict)"("Val(Sgnl)"=enum32{"Variables", "Aliases"}."Variables" ("Value (Signaling)")) -> ()  [unwired: 2 in, 2 out]
                      }
                    }
                  }
                }
              }
            }
          }
          event "VC List": Value Change {
            n228 = event-data() -> ()  [unwired: 1 in, 2 out]
            n229 = local read "VarList Mode"() -> (w544:T1)
            n230 = case shown="\"Variables\"" w544 {
              tunnel: [w547 _] -> w543
              frame "Variables" {
                n231 = property on="Var List" class="MCListbox (strict)"("Value"=i32[] [] ("Var List"), "TopLeft"=T4 {"Row"=0, "Column"=0} ("Top Left Visible Cell")) -> (error out=w547:errorcluster)  [unwired: 2 in, 1 out]
              }
              frame "Aliases" {
              }
            }
            n232 = Enqueue Element(queue=w546, element="UPDATE;", error in (no error)=w543) -> ()  [unwired: 1 in, 3 out]
          }
          event "Var List": Shortcut Menu Activation? {
            n233 = event-data() -> ("CtlRef"=w556:refnum<vi>, "MenuRef"=w555:refnum<k9>, "Coords"=w554:T16)  [unwired: 1 in]
            n234 = local read "VarList Mode"() -> (w552:T1)
            n235 = Equal?(x=w552, y=enum32{"Variables", "Aliases"}."Variables") -> (x = y?=w550:bool)
            n236 = call "VM Spy - build variable list shortcut menu.vi"("Variable List mode (T)"=w550, "Coords"=w554, "MenuRef"=w555, "CtlRef"=w556) -> ("Discard menu"=w553:bool)  [unwired: 7 in]
            n237 = event-data("Discard?"=w553) -> ()  [unwired: 1 in, 1 out]
          }
          event "Var List": Double Click {
            n238 = event-data() -> ("CtlRef"=w564:refnum<vi>, "PlatMods"=w558:T15, "Row"=w561:i32)  [unwired: 1 in, 3 out]
            n239 = Unbundle By Name(w558) -> ("Ctrl"=w557:bool)
            n240 = property on="Property Node" class="MCListbox (strict)"(reference=w564) -> ("ItemNames"=w563:string[][])  [unwired: 1 in, 2 out]
            n241 = Index Array(array=w563, index (row)=w561, index (col)=0 ("disabled index (col)")) -> (element=w559:string)
            n242 = Empty String/Path?(string/path=w559) -> (empty?=w560:bool)
            n243 = case shown="False" w560 {
              tunnel: w559 -> [w571 _]
              tunnel: w557 -> [w565 _]
              frame False {
                n244 = property on="VC List" class="MCListbox (strict)"() -> ("ItemNames"=w567:string[][], "Value"=w568:i32)  [unwired: 2 in, 2 out]
                n245 = Index Array(array=w567, index (row)=w568, index (col)=0 ("disabled index (col)")) -> (element=w570:string)
                n246 = Decimal String To Number(string=w570) -> (number=w566:i32)  [unwired: 2 in, 1 out]
                n247 = case shown="True" w565 {
                  tunnel: w571 -> [w573 w575]
                  tunnel: w566 -> [w572 w574]
                  frame False {
                    n248 = call "Inspector Launcher [VarMan Spy].vi"("VC Handle"=w572, "Variable"=w573) -> ()  [unwired: 7 in, 1 out]
                  }
                  frame True {
                    n249 = call "VM Spy - Dialog - Set Variable Value.vi"("var name"=w575, "VC Handle"=w574) -> ()  [unwired: 9 in, 1 out]
                  }
                }
              }
              frame True {
              }
            }
          }
          event "Var List": Value Change {
            n250 = event-data() -> ()  [unwired: 1 in, 6 out]
            n251 = Enqueue Element(queue=w576, element="Update Var Info;") -> ()  [unwired: 2 in, 3 out]
          }
          event "NamePtrn": Value Change {
            n252 = event-data() -> ("CtlRef"=w582:refnum<vi>, "NewVal"=w579:string)  [unwired: 1 in, 4 out]
            n253 = call <vilib>:"Trim Whitespace.vi"("string"=w579) -> ("trimmed string"=w580:string)  [unwired: 1 in]
            n254 = Not Equal?(x=w580, y=w579) -> (x != y?=w581:bool)
            n255 = case shown="True" w581 {
              tunnel: w582 -> [_ w587]
              tunnel: w580 -> [_ w586]
              tunnel: [_ w585] -> w578
              frame False {
              }
              frame True {
                n256 = property class="Str"(reference=w587, "Value"=w586) -> (error out=w585:errorcluster)  [unwired: 1 in, 1 out]
              }
            }
            n257 = Enqueue Element(queue=w583, element="Update Var List;", error in (no error)=w578) -> ()  [unwired: 1 in, 3 out]
          }
          event "EnaFilter": Value Change {
            n258 = event-data() -> ()  [unwired: 1 in, 6 out]
            n259 = Enqueue Element(queue=w588, element="Update Var List;") -> ()  [unwired: 2 in, 3 out]
          }
          event Value Change {
            n260 = event-data() -> ("NewVal"=w594:T1)  [unwired: 1 in]
            n261 = case shown="\"Aliases\"" w594 {
              tunnel: [_ w598] -> w591
              frame "Variables" {
              }
              frame "Aliases" {
                n262 = property on="VC List" class="MCListbox (strict)"("Value"=-1 ("VC List"), "TopLeft"=T4 {"Row"=0, "Column"=0} ("Top Left Visible Cell")) -> (error out=w598:errorcluster)  [unwired: 2 in, 1 out]
              }
            }
            n263 = property on="Var List" class="MCListbox (strict)"(error in=w591, "Value"=i32[] [] ("Var List"), "TopLeft"=T4 {"Row"=0, "Column"=0} ("Top Left Visible Cell")) -> (error out=w590:errorcluster)  [unwired: 1 in, 1 out]
            n264 = Enqueue Element(queue=w595, element="UPDATE;", error in (no error)=w590) -> ()  [unwired: 1 in, 3 out]
          }
          event "ctx info line": Shortcut Menu Activation? {
            n265 = event-data() -> ("MenuRef"=w615:refnum<k9>, "CtlRef"=w614:refnum<vi>)  [unwired: 1 in]
            n266 = property class="Str"(reference=w614) -> ("Value"=w609:string)  [unwired: 1 in, 2 out]
            n267 = property on="VC List" class="MCListbox (strict)"() -> ("Value"=w604:i32)  [unwired: 2 in, 2 out]
            n268 = Less Than 0?(x=w604) -> (x < 0?=w601:bool)
            n269 = Match Pattern(string=w609, regular expression="\\.[Vv][Ii]$") -> (offset past match=w606:i32)  [unwired: 1 in, 3 out]
            n270 = Less Than 0?(x=w606) -> (x < 0?=w605:bool)
            n271 = Select(t="DIS", s=w601, f="") -> (s? t:f=w600:string)
            n272 = Select(t="DIS", s=w605, f="") -> (s? t:f=w610:string)
            n273 = Format Into String(format string="Context info...          : spy_vc_info    : %s\n-\nOpen VI                     : spy_vc_open_vi : %s", w600, w610) -> (resulting string=w607:string)  [unwired: 2 in, 1 out]
            n274 = call "[ce] Create menu at runtime.vi"("menu descriptor"=w607, "menu"=w615) -> ()  [unwired: 8 in, 2 out]
            n275 = event-data() -> ()  [unwired: 2 in, 1 out]
          }
        }
      }
      frame "STARTUP" {
        n276 = Concatenate Strings("Reset Controls;\nRW INI File = LOAD;\n\nINIT;", w618) -> (w617:string)
      }
      frame "INIT" {
        n277 = Enqueue Element(queue=w620, element="UPDATE = 0;") -> ()  [unwired: 2 in, 3 out]
        n278 = invoke class="VI" method="FP.Open"("Activate"=TRUE ("Activate?"), "State"=T12."Standard") -> ()  [unwired: 3 in, 5 out]
        n279 = Concatenate Strings("", w625) -> (w624:string)
      }
      frame "RW INI File" {
        n280 = Equal?(x=w642, y="SAVE") -> (x = y?=w640:bool)
        n281 = control-ref of="This VI"() -> (w626:refnum<vi>)
        n282 = call <vilib>:"Open Config Data.vi"("configuration file path"=w643) -> ("error out"=w638:errorcluster, "refnum"=w639:T18)  [unwired: 8 in, 1 out]
        n283 = Select(t=enum16{"load", "save"}."save" ("cmd (load)"), s=w640, f=enum16{"load", "save"}."load" ("cmd (load)")) -> (s? t:f=w631:enum16{"load", "save"})
        n284 = control-ref of="VarList Mode"() -> (w630:refnum<vi>)
        n285 = control-ref of="EnaFilter"() -> (w629:refnum<vi>)
        n286 = control-ref of="NamePtrn"() -> (w628:refnum<vi>)
        n287 = call "[ce] INI - RW FP Window Position & Size.vi"("cmd (load)"=w631, "error in"=w638, "VI Refnum"=w626, "INI refnum"=w639) -> ("error out"=w633:errorcluster, "dup INI refnum"=w635:T18)  [unwired: 4 in, 2 out]
        n288 = Build Array(w630, w629, w628) -> (w627:refnum<vi>[])
        n289 = call "[ce] INI - RW Control Values.vi"("cmd (load)"=w631, "error in"=w633, "Ctrl refnums"=w627, "INI refnum"=w635) -> ("error out"=w632:errorcluster, "dup INI refnum"=w634:T18)  [unwired: 6 in]
        n290 = control-ref of="Var List"() -> (w646:refnum<vi>)
        n291 = control-ref of="VC List"() -> (w647:refnum<vi>)
        n292 = call "[ce] INI - RW MCList Properties.vi"("cmd (load)"=w631, "error in"=w632, "MCListbox Refnum"=w647, "INI refnum"=w634) -> ("error out"=w645:errorcluster, "dup INI refnum"=w649:T18)  [unwired: 6 in]
        n293 = call "[ce] INI - RW MCList Properties.vi"("cmd (load)"=w631, "error in"=w645, "MCListbox Refnum"=w646, "INI refnum"=w649) -> ("error out"=w644:errorcluster, "dup INI refnum"=w648:T18)  [unwired: 6 in]
        n294 = call <vilib>:"Close Config Data.vi"("error in (no error)"=w644, "refnum"=w648) -> ()  [unwired: 8 in, 2 out]
      }
      frame "EXIT" {
        n295 = Enqueue Element(queue=w651, element="EXIT;") -> ()  [unwired: 2 in, 3 out]
        n296 = Format Into String(format string="RW INI File = SAVE;\nReset Controls;\n\nHALT = %s;", w654) -> (resulting string=w653:string)  [unwired: 2 in, 1 out]
      }
      frame "HALT" {
        n297 = case shown="Default" w656 {
          frame "KeepFPOpen" {
          }
          frame Default {
            n298 = invoke class="VI" method="FP.Close"() -> ()  [unwired: 3 in, 3 out]
          }
        }
      }
      frame "------------------------------------ 1" {
      }
      frame "Reset Controls" {
        w662 = i32[] [] ("Item Symbols")
        w663 = string[][] [] ("Item Names")
        w664 = T4 {"Row"=0, "Column"=0} ("Top Left Visible Cell")
        n299 = property on="VC List" class="MCListbox (strict)"("Value"=-1 ("VC List"), "TopLeft"=w664, "ItemNames"=w663, "ItemSyms"=w662) -> ()  [unwired: 2 in, 2 out]
        n300 = local write "VarList Mode"(VM_Spy_Type_-_Display_Mode_Selector."Variables" ("VarList Mode")) -> ()
        n301 = property on="Var List" class="MCListbox (strict)"("Value"=i32[] [] ("Var List"), "TopLeft"=w664, "ItemNames"=w663, "ItemSyms"=w662) -> ()  [unwired: 2 in, 2 out]
      }
      frame "Menu" {
        n302 = property on="Var List" class="MCListbox (strict)"() -> ("ItemNames"=w675:string[][], "Value"=w670:i32[])  [unwired: 2 in, 2 out]
        n303 = call "[ce] State Queue Parser.vi"("input queue"=w684) -> ("state parameters"=w668:string, "state"=w677:string)  [unwired: 6 in, 1 out]
        n304 = property on="VC List" class="MCListbox (strict)"() -> ("ItemNames"=w679:string[][], "Value"=w680:i32)  [unwired: 2 in, 2 out]
        n305 = Index Array(array=w670) -> (element=w673:i32)  [unwired: 1 in]
        n306 = Index Array(array=w675, index (col)=0 ("disabled index (col)")) -> (element=w671:string[])  [unwired: 1 in]
        n307 = Index Array(array=w679, index (row)=w680, index (col)=0 ("disabled index (col)")) -> (element=w682:string)
        n308 = Index Array(array=w671, index=w673) -> (element=w672:string)
        n309 = Decimal String To Number(string=w682) -> (number=w676:i32)  [unwired: 2 in, 1 out]
        n310 = case shown="\"Refresh\"" w677 {
          selector: w677 -> [w692 _ _ _ _ _ _ _ _ _ _ _ _ _ _ _ _ _ _ _ _ _ _]
          tunnel: [_ w695 TRUE ("Assigned") w706 w708 w710 _ TRUE w725 w739 _ w750 w756 w762 _ _ _ _ _ _ TRUE _ _] -> w678
          tunnel: [_ _ _ _ _ _ _ _ _ _ _ _ _ _ _ _ _ _ _ _ _ _ "EXIT;"] -> w683
          tunnel: w676 -> [_ _ _ w705 w707 w709 _ _ w729 w738 w745 w752 w755 w764 _ _ _ _ _ _ _ _ _]
          tunnel: w672 -> [_ _ _ _ _ _ _ w724 _ _ _ w751 w754 w763 _ _ _ _ _ _ _ _ _]
          tunnel: w671 -> [_ _ _ _ _ _ _ _ _ w737 w744 _ _ _ _ _ _ _ _ _ _ _ _]
          tunnel: w670 -> [_ _ _ _ _ _ _ _ _ w736 w743 _ _ _ _ _ _ _ _ _ _ _ _]
          tunnel: w668 -> [_ _ _ _ _ _ _ _ _ _ _ _ _ _ _ _ _ _ _ _ _ w798 _]
          tunnel: [_ _ w698 _ _ _ _ w719 w726 _ _ _ "UPDATE;\nUpdate Var Info;" "UPDATE;\nUpdate Var Info;" _ _ _ _ _ _ "Update Var Info;" _ _] -> w667
          frame "", Default {
            n311 = One Button Dialog(message=w692) -> ()  [unwired: 1 in, 1 out]
          }
          frame "spy_init" {
            n312 = stacked-sequence {
              tunnel: "Initializing will close all variable contexts.\n\nDo you really want to initialize VarMan?" ("message") -> [w696]
              tunnel: [w696] -> w693
              frame #0 {
                n313 = call <vilib>:"Beep.vi"() -> ()  [unwired: 12 in]
              }
            }
            n314 = Two Button Dialog(message=w693) -> (T button?=w695:bool)  [unwired: 2 in]
            n315 = case shown="True" w695 {
              frame False {
              }
              frame True {
                n316 = call "VM - Initializing.vi"() -> ()  [unwired: 10 in, 2 out]
              }
            }
          }
          frame "spy_vc_create" {
            n317 = call "VM Spy - create context.vi"() -> ("OK out"=w700:bool, "VC Handle out"=w699:T6)  [unwired: 10 in]
            n318 = case shown="True" w700 {
              tunnel: w699 -> [_ w703]
              tunnel: [_ w701] -> w698
              frame False {
              }
              frame True {
                n319 = Format Into String(format string="UPDATE;\nHighlight Context = %d;", w703) -> (resulting string=w701:string)  [unwired: 2 in, 1 out]
                n320 = property on="VarList Mode" class="RadioBtnsControl (strict)"("Value"=enum32{"Variables", "Aliases"}."Variables" ("VarList Mode")) -> ()  [unwired: 2 in, 2 out]
              }
            }
          }
          frame "spy_vc_close" {
            n321 = call "VM Spy - close context.vi"("VC Handle"=w705) -> ("OK out"=w706:bool)  [unwired: 10 in]
          }
          frame "spy_vc_info" {
            n322 = call "VM Spy - Dialog - Context Info.vi"("VC Handle"=w707) -> ("update"=w708:bool)  [unwired: 10 in]
          }
          frame "spy_vc_name" {
            n323 = call "VM Spy - Dialog - Context Name.vi"("VC Handle"=w709) -> ("OK out"=w710:bool)  [unwired: 9 in, 1 out]
          }
          frame "spy_vc_open_vi" {
            n324 = local read "ctx info line"() -> (w713:string)
            n325 = Open VI Reference(vi path=w713) -> (vi reference=w715:refnum<vi>, error out=w717:errorcluster)  [unwired: 5 in]
            n326 = invoke class="VI" method="FP.Open"(reference=w715, error in=w717, "State"=T12."Standard") -> (reference out=w714:refnum<vi>, error out=w716:errorcluster)  [unwired: 2 in, 3 out]
            n327 = Close Reference(reference=w714, error in (no error)=w716) -> (error out=w711:errorcluster)
            n328 = call <vilib>:"Simple Error Handler.vi"("error in (no error)"=w711) -> ()  [unwired: 4 in, 5 out]
          }
          frame "spy_var_find" {
            n329 = call "VM - Variable Info.vi"("name_spec"=w724) -> ("var name"=w722:string, "var VC Handle"=w720:T6)  [unwired: 5 in, 4 out]
            n330 = property on="VarList Mode" class="RadioBtnsControl (strict)"("Value"=enum32{"Variables", "Aliases"}."Variables" ("VarList Mode")) -> ()  [unwired: 2 in, 2 out]
            n331 = Format Into String(format string="Highlight Context = %d;\nHighlight Variable = %s;\nUpdate Var Info;", w720, w722) -> (resulting string=w719:string)  [unwired: 2 in, 1 out]
          }
          frame "spy_var_create" {
            n332 = call "VM Spy - Dialog - Create variable.vi"("VC Handle"=w729) -> ("OK out"=w728:bool, "var name"=w727:string)  [unwired: 8 in, 1 out]
            n333 = case shown="True" w728 {
              tunnel: w727 -> [_ w733]
              tunnel: [_ w731] -> w726
              tunnel: [_ TRUE] -> w725
              frame False {
              }
              frame True {
                n334 = property on="VarList Mode" class="RadioBtnsControl (strict)"("Value"=enum32{"Variables", "Aliases"}."Variables" ("VarList Mode")) -> ()  [unwired: 2 in, 2 out]
                n335 = Format Into String(format string="UPDATE;\nHighlight Variable = %s;\nUpdate Var Info;", w733) -> (resulting string=w731:string)  [unwired: 2 in, 1 out]
              }
            }
          }
          frame "spy_var_destroy" {
            n336 = for {
              tunnel: w737 -> [w742]
              tunnel: w736 -> [w741] mode=indexing
              tunnel: [w740] -> w735 mode=indexing
              n337 = Index Array(array=w742, index=w741) -> (element=w740:string)
            }
            n338 = call "VM Spy - destroy variables.vi"("Var Names"=w735, "VC Handle"=w738) -> ("update"=w739:bool)  [unwired: 9 in]
          }
          frame "spy_var_inspect" {
            n339 = for {
              tunnel: w745 -> [w749]
              tunnel: w744 -> [w748]
              tunnel: w743 -> [w746] mode=indexing
              n340 = Index Array(array=w748, index=w746) -> (element=w747:string)
              n341 = call "Inspector Launcher [VarMan Spy].vi"("VC Handle"=w749, "Variable"=w747) -> ()  [unwired: 7 in, 1 out]
            }
          }
          frame "spy_var_assign" {
            n342 = call "VM Spy - Dialog - Set Variable Value.vi"("var name"=w751, "VC Handle"=w752) -> ("Assigned"=w750:bool)  [unwired: 9 in]
          }
          frame "spy_var_history" {
            n343 = call "VHistory - History Info.vi"("VC Handle"=w755, "name_spec"=w754) -> ("valid history"=w760:bool, "dup name_spec"=w757:string)  [unwired: 5 in, 3 out]
            n344 = call "VM Spy - Dialog - History Info.vi"("var name"=w757, "vc handle"=w755) -> ("dup var name"=w758:string)  [unwired: 7 in]
            n345 = call "VHistory - History Info.vi"("VC Handle"=w755, "name_spec"=w758) -> ("valid history"=w759:bool)  [unwired: 5 in, 4 out]
            n346 = Exclusive Or(1:w760, 2:w759) -> (0:w756:bool)
          }
          frame "spy_alias_info" {
            n347 = call "VM Spy - Dialog - Alias Info.vi"("var name"=w763, "vc handle"=w764) -> ("cancel out"=w765:bool)  [unwired: 9 in]
            n348 = Not(x=w765) -> (.not. x?=w762:bool)
          }
          frame "spy_tools_isp" {
            n349 = call "[ce] CE component paths.vi"("kind of path"=[ce]_CE_component_paths_-_Kind_of_Path_Enum."Project", "append path"="CSE ISP.vi") -> ("path out"=w770:path)
            n350 = Open VI Reference(vi path=w770) -> (vi reference=w772:refnum<vi>, error out=w773:errorcluster)  [unwired: 5 in]
            n351 = invoke class="VI" method="Run VI"(reference=w772, error in=w773, "Wait until done"=FALSE ("Wait Until Done")) -> (reference out=w774:refnum<vi>)  [unwired: 2 in, 4 out]
            n352 = invoke class="VI" method="FP.Open"(reference=w774, "State"=T12."Standard") -> (reference out=w769:refnum<vi>)  [unwired: 3 in, 4 out]
            n353 = Close Reference(reference=w769) -> ()  [unwired: 1 in, 1 out]
          }
          frame "spy_tools_exnav" {
            n354 = call "[ce] CE component paths.vi"("kind of path"=[ce]_CE_component_paths_-_Kind_of_Path_Enum."Project", "append path"="CE Examples Navigator.vi") -> ("path out"=w779:path)
            n355 = Open VI Reference(vi path=w779) -> (vi reference=w781:refnum<vi>, error out=w782:errorcluster)  [unwired: 5 in]
            n356 = invoke class="VI" method="Run VI"(reference=w781, error in=w782, "Wait until done"=FALSE ("Wait Until Done")) -> (reference out=w783:refnum<vi>)  [unwired: 2 in, 4 out]
            n357 = invoke class="VI" method="FP.Open"(reference=w783, "State"=T12."Standard") -> (reference out=w778:refnum<vi>)  [unwired: 3 in, 4 out]
            n358 = Close Reference(reference=w778) -> ()  [unwired: 1 in, 1 out]
          }
          frame "spy_help_vm" {
            n359 = call "[ce] CE component paths.vi"("kind of path"=[ce]_CE_component_paths_-_Kind_of_Path_Enum."Help", "append path"="varman.hlp") -> ("path out"=w787:path)
            n360 = Control Online Help(2:w787, 3:"VarMan Overview" ("String to search for"), 4:enum16{"Contents", "Key", "Close"}."Key" ("Operation")) -> ()  [unwired: 1 in, 1 out]
          }
          frame "spy_help_spy" {
            n361 = call "[ce] CE component paths.vi"("kind of path"=[ce]_CE_component_paths_-_Kind_of_Path_Enum."Help", "append path"="varman.hlp") -> ("path out"=w792:path)
            n362 = Control Online Help(2:w792, 3:"VarMan Spy" ("String to search for"), 4:enum16{"Contents", "Key", "Close"}."Key" ("Operation")) -> ()  [unwired: 1 in, 1 out]
          }
          frame "spy_about_spy" {
            n363 = call "[ce] MsgBox - About CalcExpress.vi"("custom title"="About VarMan Spy", "message before..."="VarMan Spy utility\n") -> ()  [unwired: 9 in, 1 out]
          }
          frame "spy_about_ce" {
            n364 = call "[ce] MsgBox - About CalcExpress.vi"() -> ()  [unwired: 11 in, 1 out]
          }
          frame "Refresh" {
          }
          frame "HELP" {
            n365 = Match Pattern(string=w798, regular expression="@") -> (before substring=w805:string, after substring=w800:string)  [unwired: 1 in, 2 out]
            n366 = Empty String/Path?(string/path=w805) -> (empty?=w804:bool)
            n367 = call "[ce] CE component paths.vi"("kind of path"=[ce]_CE_component_paths_-_Kind_of_Path_Enum."Help", "append path"=w800) -> ("path out"=w799:path)
            n368 = Select(t=enum16{"Contents", "Key", "Close"}."Contents", s=w804, f=enum16{"Contents", "Key", "Close"}."Key" ("Operation")) -> (s? t:f=w801:enum16{"Contents", "Key", "Close"})
            n369 = Control Online Help(2:w799, 3:w805, 4:w801) -> ()  [unwired: 1 in, 1 out]
          }
          frame "EXIT", "spy_exit" {
          }
        }
        n370 = case shown="True" w678 {
          tunnel: w669 -> [_ w691]
          tunnel: w667 -> [_ w687]
          frame False {
          }
          frame True {
            n371 = Empty String/Path?(string/path=w687) -> (empty?=w688:bool)
            n372 = Select(t="UPDATE;" ("element"), s=w688, f=w687) -> (s? t:f=w689:string)
            n373 = Enqueue Element(queue=w691, element=w689) -> ()  [unwired: 2 in, 3 out]
          }
        }
        n374 = Concatenate Strings(w683, w686) -> (w685:string)
      }
    }
  }
